vi "Configure All.vi"(1 "RT Data in":T1={"Device ref"=0, "Scan Period (uSec)"=10000, "Device Channels"={"Status"={"BD Refs"=[], "Length"=0, "FIFO Index"=0, "Data"=[]}, "Command"={"BD Refs"=[], "Data"=[], "Length"=0, "FIFO Index"=0}}, "Local Chassis"=[], "EtherCAT Masters"=[], "Async"={"Status"=refnum, "Command"=refnum, "Input FIFO"=refnum, "Input FIFO buffer"=[], "Output FIFO"=refnum, "Output FIFO buffer"=[], "Async VI Ref"=refnum}, "ECAT Reconfig"={"Reconfig Module Found"=FALSE, "VI Ref"=refnum, "Status"=refnum}, "Device Error"={"status"=FALSE, "code"=0, "source"=""}, "DeviceName"="", "PCLSync?"=FALSE} {"Device Channels"."Status"."BD Refs"."Data Reference" format="%.0x"; "Device Channels"."Command"."BD Refs"."Data Reference" format="%.0x"; "Local Chassis"."FPGA"."VS ref" format="%.0x"; "Local Chassis"."RSI Modules"."VS ref" format="%.0x"; "Local Chassis"."VS ref" format="%.0x"; "Device ref" format="%.0x"; "EtherCAT Masters"."REM IO ECAT Slaves"."VS ref" format="%.0x"; "EtherCAT Masters"."Generic EtherCAT Slaves"."VS ref" format="%.0x"; "EtherCAT Masters"."VS ref" format="%.0x"; "EtherCAT Masters"."EtherCAT Slaves"."FPGA"."VS ref" format="%.0x"; "EtherCAT Masters"."EtherCAT Slaves"."RSI Modules"."VS ref" format="%.0x"; "EtherCAT Masters"."EtherCAT Slaves"."VS ref" format="%.0x"}) -> (0 "RT Data out":T1={"Device ref"=0, "Scan Period (uSec)"=10000, "Device Channels"={"Status"={"BD Refs"=[], "Length"=0, "FIFO Index"=0, "Data"=[]}, "Command"={"BD Refs"=[], "Data"=[], "Length"=0, "FIFO Index"=0}}, "Local Chassis"=[], "EtherCAT Masters"=[], "Async"={"Status"=refnum, "Command"=refnum, "Input FIFO"=refnum, "Input FIFO buffer"=[], "Output FIFO"=refnum, "Output FIFO buffer"=[], "Async VI Ref"=refnum}, "ECAT Reconfig"={"Reconfig Module Found"=FALSE, "VI Ref"=refnum, "Status"=refnum}, "Device Error"={"status"=FALSE, "code"=0, "source"=""}, "DeviceName"="", "PCLSync?"=FALSE} {"Device Channels"."Status"."BD Refs"."Data Reference" format="%.0x"; "Device Channels"."Command"."BD Refs"."Data Reference" format="%.0x"; "Local Chassis"."FPGA"."VS ref" format="%.0x"; "Local Chassis"."RSI Modules"."VS ref" format="%.0x"; "Local Chassis"."VS ref" format="%.0x"; "Device ref" format="%.0x"; "EtherCAT Masters"."REM IO ECAT Slaves"."VS ref" format="%.0x"; "EtherCAT Masters"."Generic EtherCAT Slaves"."VS ref" format="%.0x"; "EtherCAT Masters"."VS ref" format="%.0x"; "EtherCAT Masters"."EtherCAT Slaves"."FPGA"."VS ref" format="%.0x"; "EtherCAT Masters"."EtherCAT Slaves"."RSI Modules"."VS ref" format="%.0x"; "EtherCAT Masters"."EtherCAT Slaves"."VS ref" format="%.0x"})   [LabVIEW 2020, in "SEECD Engine.lvlib"]
uses:
  SEECD Engine.lvlib
  Includes/Modules.lvlibp/RSI Module/RSI Module.lvclass
  Type Defs/ECAT Module Reconfig.ctl
  <vilib>/NI VeriStand/Custom Device API/Custom Device Item Ref.ctl
  <vilib>/NI VeriStand/Custom Device API/Custom Device API.lvlib
  <vilib>/NI VeriStand/Custom Device API/Data Reference.ctl
  <vilib>/NI VeriStand/Custom Device API/Block Data Reference.ctl
  Type Defs/Input Data.ctl
  Type Defs/Output Data.ctl
  Type Defs/RSI Module Data.ctl
  Type Defs/FPGA Data.ctl
  Type Defs/Local Chassis Data.ctl
  Type Defs/EtherCAT Slave Data.ctl
  Type Defs/EtherCAT Master Data.ctl
  Type Defs/RT Data.ctl
  Includes/Modules.lvlibp/RSI Module/Channel Type.ctl
  Type Defs/Async Command.ctl
  Type Defs/Async Status.ctl
  Type Defs/Async State.ctl
  Shared/Type Defs/UDV Data Type.ctl
  Shared/SEECD Shared.lvlib
  Shared/Type Defs/FXP Config.ctl
  Type Defs/UDV Data.ctl
  Includes/Modules.lvlibp/RSI Module/Module Models.ctl
  Type Defs/Module Config Data.ctl
  Type Defs/Async Data.ctl
  Type Defs/ECAT Reconfig State.ctl
  Type Defs/ECAT Reconfig Status.ctl
  Type Defs/ECAT Reconfig Data.ctl
  Type Defs/Device Channels.ctl
  Type Defs/Mixed IO.ctl
  Type Defs/Open Module IOVs.ctl
  Type Defs/Mod Size Indexes.ctl
  Type Defs/Generic ECAT Slave IOV Cluster.ctl
  Type Defs/Generic ECAT Slave Data Cluster.ctl
  Type Defs/Generic ECAT Slave RT-Data-Array.ctl
  Type Defs/REM IO ECAT Slave IOV Cluster.ctl
  Type Defs/REM IO ECAT Slave Data Cluster.ctl
  Type Defs/REM IO ECAT Slave RT-Data-Array.ctl
types:
  T1 = typedef "SEECD Engine.lvlib/RT Data.ctl" = cluster{"Device ref":T2, "Scan Period (uSec)":u32, "Device Channels":T3, "Local Chassis":T8[], "EtherCAT Masters":T20[], "Async":T28, "ECAT Reconfig":T29, "Device Error":errorcluster, "DeviceName":string, "PCLSync?":bool}
  T2 = typedef "Custom Device API.lvlib/Custom Device Item Ref.ctl" = u64
  T3 = typedef "SEECD Engine.lvlib/Device Channels.ctl" = cluster{"Status":T4, "Command":T7}
  T4 = typedef "SEECD Engine.lvlib/Output Data.ctl" = cluster{"BD Refs":T5[], "Length":i32, "FIFO Index":i32, "Data":dbl[]}
  T5 = typedef "Custom Device API.lvlib/Block Data Reference.ctl" = cluster{"Data Reference":T6, "Offset":u64, "Length":u64}
  T6 = typedef "Custom Device API.lvlib/Data Reference.ctl" = i32
  T7 = typedef "SEECD Engine.lvlib/Input Data.ctl" = cluster{"BD Refs":T5[], "Data":dbl[], "Length":i32, "FIFO Index":i32}
  T8 = typedef "SEECD Engine.lvlib/Local Chassis Data.ctl" = cluster{"VS ref":T2, "RSI Modules":T9[], "FPGA":T15[], "Input Mod Size Idxs":T19, "Output Modules":i32[], "MixedIO Mod Size Idxs":T19}
  T9 = typedef "SEECD Engine.lvlib/RSI Module Data.ctl" = cluster{"VS ref":T2, "IOV ref":refnum<k21>, "Open Mod refs":T10, "Module DVR":refnum<data-value>, "Slot":u32, "Model":T11, "Channel Type":T12, "EtherCAT?":bool, "CDInput Data":T7, "CDOutput Data":T4, "Module Config Data":T13, "Mixed IO":T14}
  T10 = typedef "SEECD Engine.lvlib/Open Module IOVs.ctl" = cluster{"Analog Read":refnum<k21>, "Digital Read":refnum<k21>, "Analog Write":refnum<k21>, "Digital Write":refnum<k21>}
  T11 = typedef "Modules.lvlibp/RSI Module.lvclass/Module Models.ctl" = enum16{"Empty", "NI 9201", "NI 9203", "NI 9205", "NI 9206", "NI 9207", "NI 9208", "NI 9209", "NI 9210", "NI 9211", "NI 9212", "NI 9213", "NI 9214", "NI 9215", "NI 9216", "NI 9217", "NI 9219", "NI 9220", "NI 9221", "NI 9222", "NI 9223", "NI 9224", "NI 9225", "NI 9226", "NI 9227", "NI 9228", "NI 9229", "NI 9233", "NI 9234", "NI 9235", "NI 9236", "NI 9237", "NI 9239", "NI 9242", "NI 9244", "NI 9253", "NI 9263", "NI 9264", "NI 9265", "NI 9266", "NI 9269", "NI 9344", "NI 9350", "NI 9375", "NI 9401", "NI 9402", "NI 9403", "NI 9411", "NI 9421", "NI 9422", "NI 9423", "NI 9425", "NI 9426", "NI 9435", "NI 9436", "NI 9437", "NI 9472", "NI 9474", "NI 9475", "NI 9476", "NI 9477", "NI 9478", "NI 9481", "NI 9482", "NI 9485"}
  T12 = typedef "Modules.lvlibp/RSI Module.lvclass/Channel Type.ctl" = enum16{"Analog", "Digital"}
  T13 = typedef "SEECD Engine.lvlib/Module Config Data.ctl" = cluster{"Configurable?":bool, "Config Block Data Refs":T5[], "Config Data DVR":refnum<data-value>, "Previous Values":dbl[], "Local Reconfig VI Ref":refnum<vi>}
  T14 = typedef "SEECD Engine.lvlib/Mixed IO.ctl" = cluster{"Input Channel Indices":i32[], "Input Buffer":dbl[]}
  T15 = typedef "SEECD Engine.lvlib/FPGA Data.ctl" = cluster{"VS ref":T2, "IOV ref":refnum<k21>, "FPGA Target":enum16{"Local", "EtherCAT"}, "Product Code":u32, "Bitfile Signature":string, "Bitfile Path (RT)":path, "FPGA Session":u32, "Input Data":T7, "Output Data":T4, "UDVs":cluster{"From FPGA":T16[], "To FPGA":T16[]}}
  T16 = typedef "SEECD Engine.lvlib/UDV Data.ctl" = cluster{"VS ref":T2, "IOV Ref":refnum<k21>, "Name":string, "UDV Data Type":T17, "Supported Type?":bool, "FXP Config":T18, "FXP VI Ref":refnum<vi>}
  T17 = typedef "SEECD Shared.lvlib/UDV Data Type.ctl" = enum16{"Boolean", "Fixed Point", "Int8", "Int16", "Int32", "Int64", "U32 Bit Field", "UInt8", "UInt16", "UInt32", "UInt64", "Other", "DBL", "SGL"}
  T18 = typedef "SEECD Shared.lvlib/FXP Config.ctl" = cluster{"signed":bool, "size":u32, "integersize":i32}
  T19 = typedef "SEECD Engine.lvlib/Mod Size Indexes.ctl" = cluster{"4":i32[], "8":i32[], "16":i32[], "32":i32[], "other":i32[]}
  T20 = typedef "SEECD Engine.lvlib/EtherCAT Master Data.ctl" = cluster{"VS ref":T2, "IOV ref":refnum<k21>, "Master ID":u32, "Cyclic Data Bandwidth":u32, "EtherCAT Slaves":T21[], "Generic EtherCAT Slaves":T22, "REM IO ECAT Slaves":T25}
  T21 = typedef "SEECD Engine.lvlib/EtherCAT Slave Data.ctl" = cluster{"VS ref":T2, "IOV ref":refnum<k21>, "Position Address":u16, "RSI Modules":T9[], "FPGA":T15[], "Input Mod Size Idxs":T19, "Output Modules":i32[], "MixedIO Mod Size Idxs":T19}
  T22 = typedef "SEECD Engine.lvlib/Generic ECAT Slave RT-Data-Array.ctl" = T23[]
  T23 = typedef "SEECD Engine.lvlib/Generic ECAT Slave Data Cluster.ctl" = cluster{"VS ref":T2, "IOV ref":refnum<k21>, "Position Address":u16, "I/O Imput Vars ":T24[], "I/O Output Vars":T24[], "I/O Input Data":T7, "I/O Output Data":T4, "Distributed Clock":bool}
  T24 = typedef "SEECD Engine.lvlib/Generic ECAT Slave IOV Cluster.ctl" = cluster{"VS ref":T2, "IOV Ref":refnum<k21>, "Name":string, "UDV Data Type":T17}
  T25 = typedef "SEECD Engine.lvlib/REM IO ECAT Slave RT-Data-Array.ctl" = T26[]
  T26 = typedef "SEECD Engine.lvlib/REM IO ECAT Slave Data Cluster.ctl" = cluster{"VS ref":T2, "IOV ref":refnum<k21>, "Position Address":u16, "I/O Imput Vars ":T27[], "I/O Output Vars":T27[], "I/O Input Data":T7, "I/O Output Data":T4}
  T27 = typedef "SEECD Engine.lvlib/REM IO ECAT Slave IOV Cluster.ctl" = cluster{"VS ref":T2, "IOV Ref":refnum<k21>, "Name":string, "UDV Data Type":T17, "Scaling Factor":dbl}
  T28 = typedef "SEECD Engine.lvlib/Async Data.ctl" = cluster{"Status":refnum<queue>, "Command":refnum<queue>, "Input FIFO":refnum<k33>, "Input FIFO buffer":dbl[], "Output FIFO":refnum<k33>, "Output FIFO buffer":dbl[], "Async VI Ref":refnum<vi>}
  T29 = typedef "SEECD Engine.lvlib/ECAT Reconfig Data.ctl" = cluster{"Reconfig Module Found":bool, "VI Ref":refnum<vi>, "Status":refnum<queue>}
  T30 = typedef "SEECD Engine.lvlib/ECAT Module Reconfig.ctl" = cluster{"Module DVR":refnum<data-value>, "IOV ref":refnum<k21>, "Config Data DVR":refnum<data-value>}
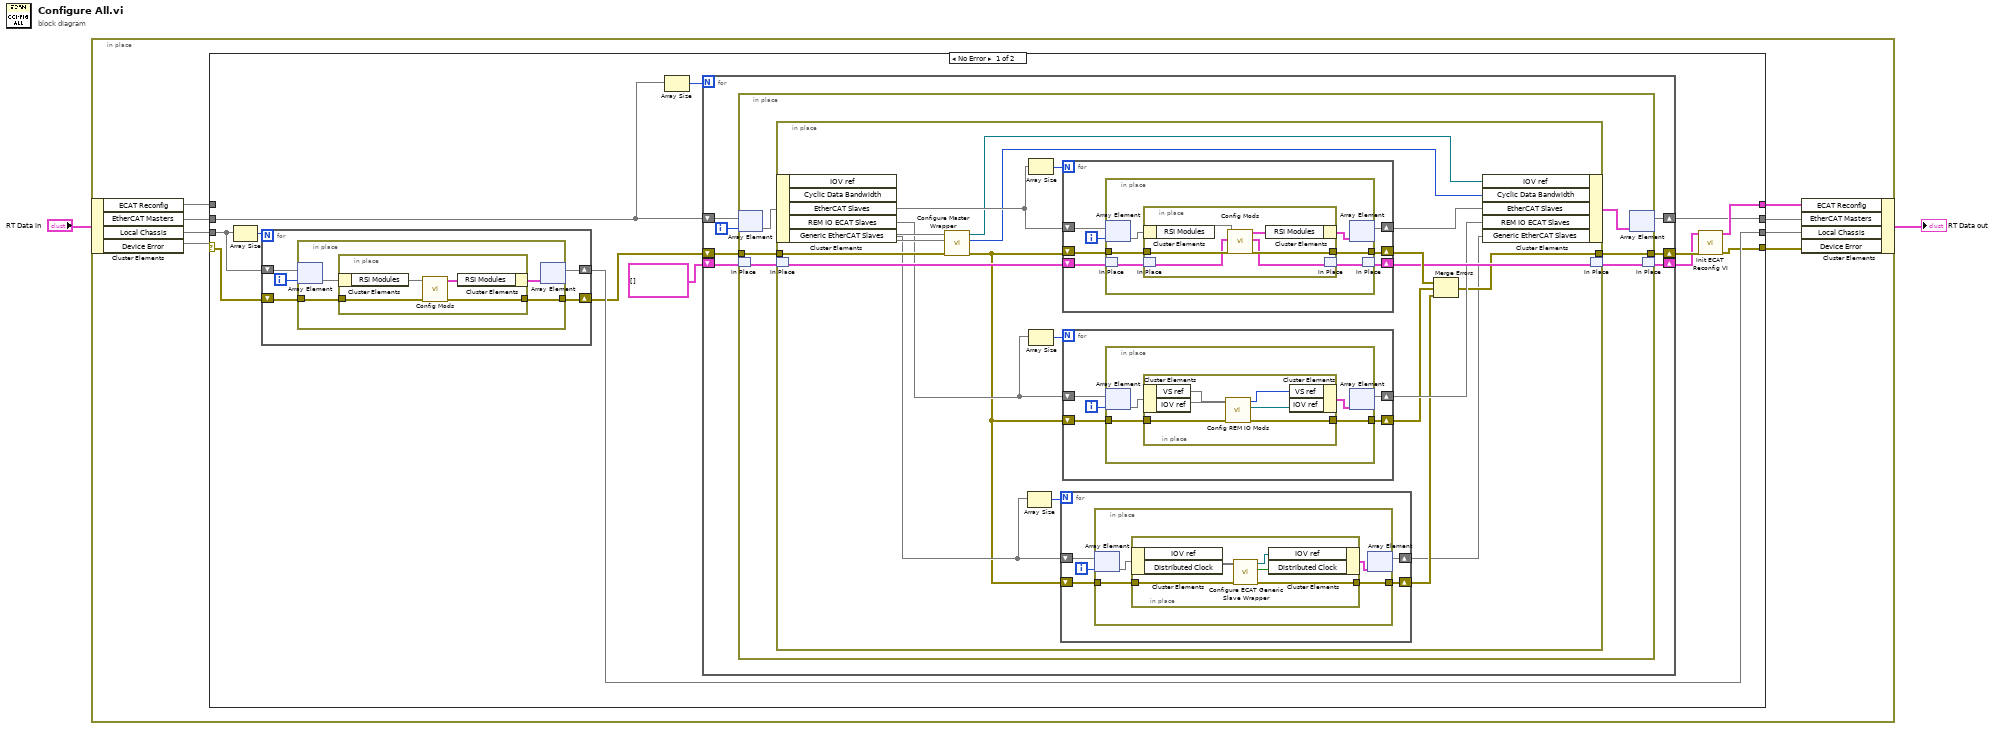
[diagram p0: block diagram]
diagram:
  n1 = in-place {
    n2 = in-place-cluster #1("RT Data in") -> ("ECAT Reconfig"=w3, "EtherCAT Masters"=w9, "Local Chassis"=w8, "Device Error"=w10)
    n3 = case shown="No Error" w10 {
      selector: w10 -> [w19 w123]
      tunnel: [w12 w123] -> w7
      tunnel: w9 -> [w22 w121]
      tunnel: w8 -> [w20 w122]
      tunnel: [w18 w122] -> w6
      tunnel: [w11 w121] -> w5
      tunnel: [w13 w120] -> w4
      tunnel: w3 -> [_ w120]
      frame No Error {
        n4 = Array Size(array=w20) -> (size(s)=w21:i32)
        n5 = for {
          N: w21 -> [_]
          shift-right: [w24] -> w18
          shift-left: w20 -> [w28]
          shift-right: [w25] -> w17
          shift-left: w19 -> [w26]
          i -> [w27]
          n6 = in-place {
            in-place-border: w26 -> [w30]
            in-place-border: [w29] -> w25
            n7 = in-place-array #2(w28, w27) -> (w32)
            n8 = in-place {
              in-place-border: w30 -> [w34]
              in-place-border: [w33] -> w29
              n9 = in-place-cluster #3(w32) -> ("RSI Modules"=w36)
              n10 = call "Config Mods.vi"("error in (no error)"=w34, "RSI Modules in"=w36) -> ("error out"=w33:errorcluster, "RSI Modules out"=w35:T9[])  [unwired: 7 in, 1 out]
              n11 = in-place-cluster #3("RSI Modules"=w35) -> (w31:cluster{})
            }
            n12 = in-place-array #2(w31) -> (w24)  [unwired: 1 out]
          }
        }
        n13 = Array Size(array=w22) -> (size(s)=w23:i32)
        n14 = for {
          N: w23 -> [_]
          shift-right: [w40] -> w15
          shift-left: w17 -> [w41]
          shift-right: [w39] -> w11
          shift-left: w22 -> [w43]
          shift-right: [w37] -> w14
          shift-left: T30[] [] -> [w38]
          i -> [w42]
          n15 = in-place {
            in-place-border: w41 -> [w48]
            in-place-border: [w47] -> w40
            n16 = in-place-array #4(w43, w42) -> (w49)
            n17 = in-place-match #5(w38) -> (w45:T30[])
            n18 = in-place {
              in-place-border: w48 -> [w64]
              in-place-border: [w56] -> w47
              n19 = in-place-cluster #6(w49) -> ("IOV ref"=w62, "Cyclic Data Bandwidth"=w63, "EtherCAT Slaves"=w70, "REM IO ECAT Slaves"=w59, "Generic EtherCAT Slaves"=w53)
              n20 = in-place-match #7(w45) -> (w66:T30[])
              n21 = call "Configure Master Wrapper.vi"("error in"=w64, "Cyclic Data Bandwidth"=w63, "IOV ref in"=w62) -> ("error out"=w50:errorcluster, "Cyclic Data Bandwidth out"=w61:u32, "IOV ref out"=w60:refnum<k21>)  [unwired: 6 in]
              n22 = Array Size(array=w53) -> (size(s)=w54:i32)
              n23 = Array Size(array=w70) -> (size(s)=w69:i32)
              n24 = Array Size(array=w59) -> (size(s)=w57:i32)
              n25 = for {
                N: w54 -> [_]
                shift-right: [w71] -> w52
                shift-left: w50 -> [w74]
                shift-right: [w73] -> w51
                shift-left: w53 -> [w72]
                i -> [w75]
                n26 = in-place {
                  in-place-border: w74 -> [w79]
                  in-place-border: [w78] -> w71
                  n27 = in-place-array #8(w72, w75) -> (w76)
                  n28 = in-place {
                    in-place-border: w79 -> [w85]
                    in-place-border: [w84] -> w78
                    n29 = in-place-cluster #9(w76) -> ("IOV ref"=w80, "Distributed Clock"=w83)
                    n30 = call "Configure ECAT Generic Slave Wrapper.vi"("error in"=w85, "Distributed Clock"=w83, "IOV ref"=w80) -> ("error out"=w84:errorcluster, "Distributed Clock out"=w82:bool, "IOV ref out"=w81:refnum<k21>)  [unwired: 6 in]
                    n31 = in-place-cluster #9("IOV ref"=w81, "Distributed Clock"=w82) -> (w77:cluster{})
                  }
                  n32 = in-place-array #8(w77) -> (w73)  [unwired: 1 out]
                }
              }
              n33 = for {
                N: w69 -> [_]
                shift-right: [w104] -> w68
                shift-left: w50 -> [w105]
                shift-right: [w103] -> w67
                shift-left: w70 -> [w107]
                shift-right: [w101] -> w65
                shift-left: w66 -> [w102]
                i -> [w106]
                n34 = in-place {
                  in-place-border: w105 -> [w112]
                  in-place-border: [w111] -> w104
                  n35 = in-place-array #10(w107, w106) -> (w113)
                  n36 = in-place-match #11(w102) -> (w109:T30[])
                  n37 = in-place {
                    in-place-border: w112 -> [w117]
                    in-place-border: [w116] -> w111
                    n38 = in-place-cluster #12(w113) -> ("RSI Modules"=w119)
                    n39 = in-place-match #13(w109) -> (w115:T30[])
                    n40 = call "Config Mods.vi"("error in (no error)"=w117, "ECAT Mod Reconfig in"=w115, "RSI Modules in"=w119) -> ("error out"=w116:errorcluster, "ECAT Mod Reconfig out"=w114:T30[], "RSI Modules out"=w118:T9[])  [unwired: 6 in]
                    n41 = in-place-cluster #12("RSI Modules"=w118) -> (w110:cluster{})
                    n42 = in-place-match #13(w114) -> (w108:T30[])
                  }
                  n43 = in-place-array #10(w110) -> (w103)  [unwired: 1 out]
                  n44 = in-place-match #11(w108) -> (w101:T30[])
                }
              }
              n45 = for {
                N: w57 -> [_]
                shift-right: [w86] -> w55
                shift-left: w50 -> [w89]
                shift-right: [w88] -> w58
                shift-left: w59 -> [w87]
                i -> [w90]
                n46 = in-place {
                  in-place-border: w89 -> [w94]
                  in-place-border: [w91] -> w86
                  n47 = in-place-array #14(w87, w90) -> (w93)
                  n48 = in-place {
                    in-place-border: w94 -> [w100]
                    in-place-border: [w99] -> w91
                    n49 = in-place-cluster #15(w93) -> ("VS ref"=w96, "IOV ref"=w98)
                    n50 = call "Config REM IO Mods.vi"("error in (no error)"=w100, "IOV Ref In"=w98, "VS Ref In"=w96) -> ("error out"=w99:errorcluster, "IOV Ref Out"=w97:refnum<k21>, "VS Ref Out"=w95:T2)  [unwired: 6 in]
                    n51 = in-place-cluster #15("VS ref"=w95, "IOV ref"=w97) -> (w92:cluster{})
                  }
                  n52 = in-place-array #14(w92) -> (w88)  [unwired: 1 out]
                }
              }
              n53 = Merge Errors(w68, w55, w52) -> (w56:errorcluster)
              n54 = in-place-cluster #6("IOV ref"=w60, "Cyclic Data Bandwidth"=w61, "EtherCAT Slaves"=w67, "REM IO ECAT Slaves"=w58, "Generic EtherCAT Slaves"=w51) -> (w46:cluster{})
              n55 = in-place-match #7(w65) -> (w44:T30[])
            }
            n56 = in-place-array #4(w46) -> (w39)  [unwired: 1 out]
            n57 = in-place-match #5(w44) -> (w37:T30[])
          }
        }
        n58 = call "Init ECAT Reconfig VI.vi"("error in (no error)"=w15, "ECAT Modules"=w14) -> ("error out"=w12:errorcluster, "ECAT Reconfig out"=w13:T29)  [unwired: 8 in]
      }
      frame Error {
      }
    }
    n59 = in-place-cluster #1("ECAT Reconfig"=w4, "EtherCAT Masters"=w5, "Local Chassis"=w6, "Device Error"=w7) -> (→"RT Data out":cluster{})
  }
